vi "get bitfiles from files array.vi"(3 "file paths":path[](array[path])) -> (1 "FPGA bitfiles":path[](array[path]))   [LabVIEW 2014]
uses:
  <vilib>/regexp/Match Regular Expression.xnode
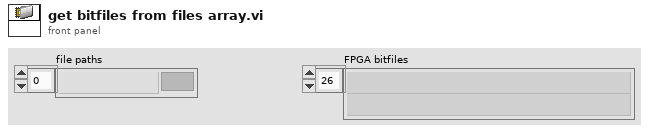
[diagram p1: front panel]
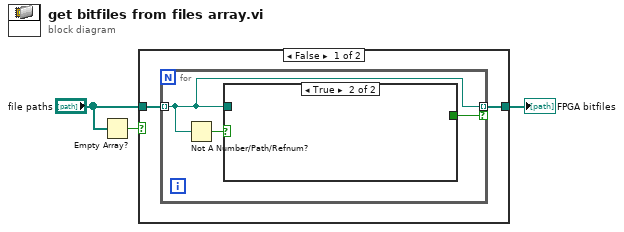
[diagram p0: block diagram]
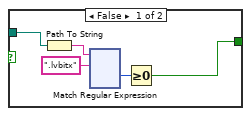
[diagram p2: hidden frame]
diagram:
  n1 = Empty Array?(array="file paths") -> (empty?=w2:bool)
  n2 = case shown="False" w2 {
    tunnel: "file paths" -> [w5 w128]
    tunnel: [w4 w128] -> w3
    frame False {
      n3 = for {
        tunnel: w5 -> [w7] mode=indexing
        tunnel: [w7] -> w4 mode=indexing if=w8
        n4 = Not A Number/Path/Refnum?(number/path/refnum=w7) -> (NaN/Path/Refnum?=w6:bool)
        n5 = case shown="True" w6 {
          tunnel: [w10 _] -> w8
          tunnel: w7 -> [w9 _]
          frame False {
            n6 = Path To String(path=w9) -> (string=w12:string)
            n7 = xnode "Match Regular Expression"("input string"=w12, "regular expression"=".lvbitx") -> ("offset past match"=w11:i32)  [unwired: 4 in, 4 out]
            n8 = Greater Or Equal To 0?(x=w11) -> (x >= 0?=w10:bool)
          }
          frame True {
          }
        }
      }
    }
    frame True {
    }
  }
  "FPGA bitfiles" <- w3
